vi "XPN Is Defect Ready.vi"(8 "error in (no error)":errorcluster, 11 "defectReady":i32) -> (0 "error out":errorcluster, 2 "function return":i32, 3 "defectReady out":i32)   [LabVIEW 2025, in "xPanelWrapper.lvlib"]
doc: "XPN_API int XPN_IsDefectReady(int* defectReady);"
uses:
  xPanelWrapper.lvlib
  xPanelWrapper.dll
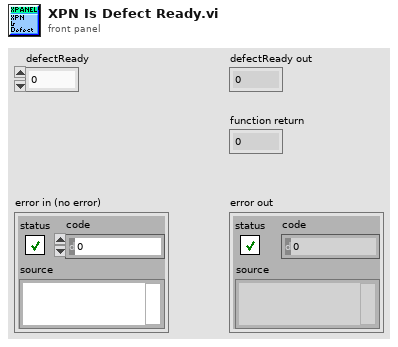
[diagram p1: front panel]
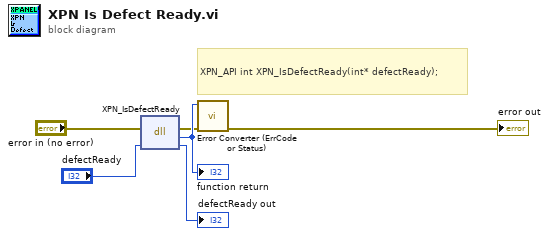
[diagram p0: block diagram]
diagram:
  # "XPN_API int XPN_IsDefectReady(int* defectReady);"
  n1 = dll-call lib="E:/GitHub/xPanelWrapper/xPanelWrapperLvLib/xPanelWrapper.*" fn="XPN_IsDefectReady"(error in="error in (no error)", "defectReady"="defectReady") -> (error out=w2:errorcluster, w6:i32, "defectReady"=→"defectReady out":i32)  [unwired: 2 in, 1 out]
  "function return" <- w6
  n2 = call "Error Converter (ErrCode or Status).vi"("error in (no error)"=w2, "error code"=w6) -> ("error out"=→"error out":errorcluster)  [unwired: 9 in]
